vi "Run Sample Metadata.vi"(0 "Image File (Path/Name)":path, 11 "Error In":errorcluster) -> (4 "Image File (Dup)":path, 15 "Error Out":errorcluster)   [LabVIEW 2016]
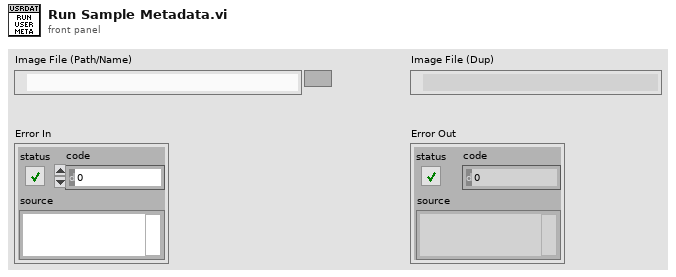
[diagram p1: front panel]
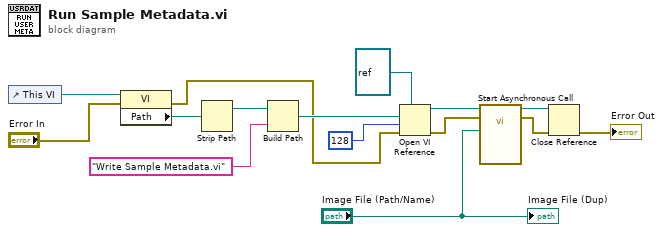
[diagram p0: block diagram]
diagram:
  n1 = control-ref of="This VI"() -> (w15:refnum<vi>)
  n2 = property class="VI"(reference=w15, error in="Error In") -> (error out=w1:errorcluster, "Path"=w14:path)  [unwired: 1 out]
  n3 = Strip Path(path=w14) -> (stripped path=w13:path)  [unwired: 1 out]
  n4 = Build Path(base path=w13, name or relative path="Write Sample Metadata.vi") -> (appended path=w11:path)
  n5 = Open VI Reference(type specifier VI Refnum (for type only)=refnum<vi> refnum, vi path=w11, options=128, error in (no error)=w1) -> (vi reference=w8:refnum<vi>, error out=w6:errorcluster)  [unwired: 2 in]
  n6 = call-by-ref "Start Asynchronous Call"(reference=w8, error in=w6, "File Path"="Image File (Path/Name)") -> (reference out=w7:refnum<vi>, error out=w5:errorcluster)  [unwired: 12 in, 3 out]
  n7 = Close Reference(reference=w7, error in (no error)=w5) -> (error out=→"Error Out":errorcluster)
  "Image File (Dup)" <- "Image File (Path/Name)"
